vi "Lithographify.vi"(0 "interpolation distance":dbl, 1 "Path Settings.lvclass":refnum<class "Path Settings.lvclass">, 5 "Data In":cluster{string, cluster{"X":dbl, "Y":dbl}[]}, 7 "Direction":u16, 9 "Speed (um/s)":T1={"Schedule"=enum."Constant", "Settings"=variant(dbl 0.0)}, 11 "Voltage (V)":T1={"Schedule"=enum."Constant", "Settings"=variant(dbl 0.0)}, 13 "Enabled":bool) -> (4 "Lithography Data":T3)   [LabVIEW 2019]
doc: "This VI calculates the lithography data of one pattern and organizes it appropriately."
uses:
  typedefs/Schedule Types/Schedule--Formula.ctl
  Classes/Settings/ObjectSettings/ObjectSettings.lvclass
  Classes/Settings/Path Settings/Path Settings.lvclass
  typedefs/Schedule - enum.ctl
  typedefs/Voltage - cluster.ctl
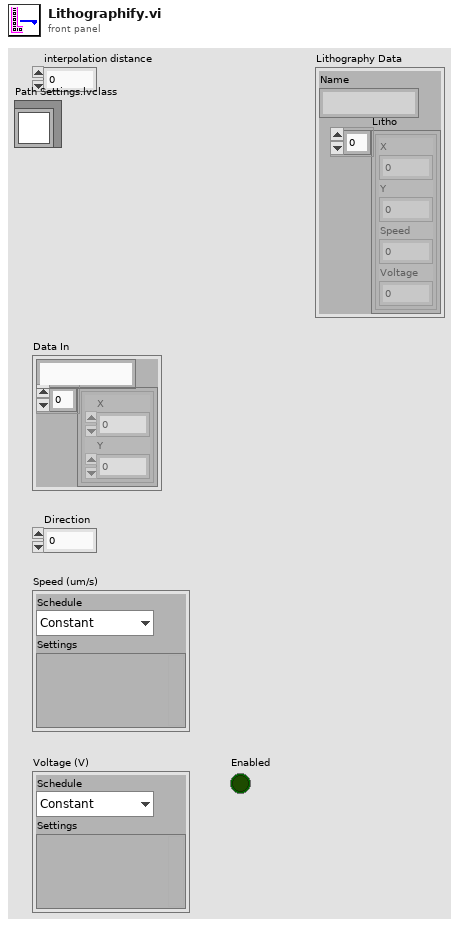
[diagram p1: front panel]
types:
  T1 = typedef "Voltage - cluster.ctl" = cluster{"Schedule":T2, "Settings":variant}
  T2 = typedef "Schedule - enum.ctl" = enum16{"Constant", "Ramp", "Fn. Generator", "Formula"}
  T3 = cluster{"Name":string, "Litho":cluster{"X":dbl, "Y":dbl, "Speed":dbl, "Voltage":dbl}[]}
  T4 = cluster{"X":dbl, "Y":dbl, "Speed":dbl, "Voltage":dbl}[]
  T5 = cluster{"X":dbl, "Y":dbl, "Speed":dbl, "Voltage":dbl}
  T6 = typedef "Schedule--Formula.ctl" = cluster{"formula":string, "formula length (nm)":dbl, "formula resolution (nm)":dbl}
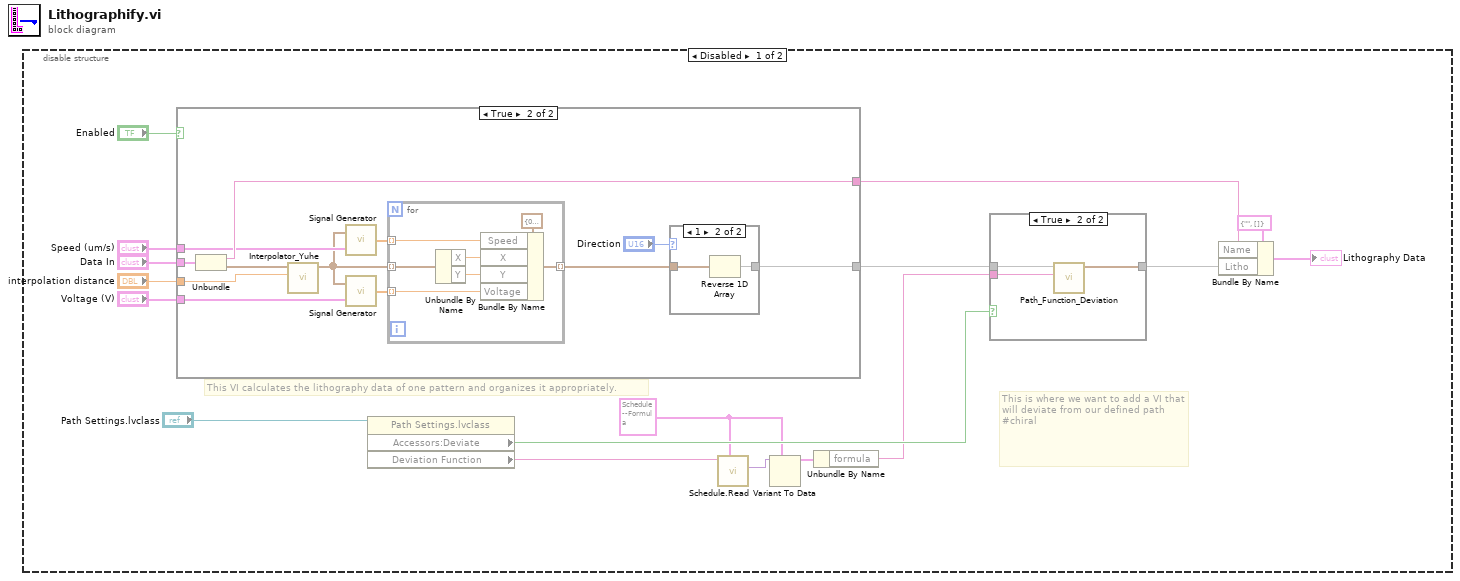
[diagram p0: block diagram]
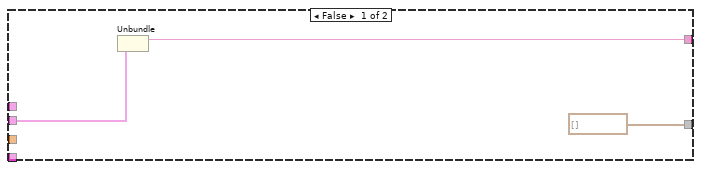
[diagram p3: hidden frame]
diagram:
  n1 = disable-structure shown="Disabled" {
    frame Disabled {
      w5 = T6 {"formula"="1*(step(170-t)*cos(0.62831853071*t)+step(t-170)*cos(0.62831853071*(t-170))*(-1))", "formula length (nm)"=340.0, "formula resolution (nm)"=0.001} ("Formula")
      # "This is where we want to add a VI that will deviate from our defined path\n#chiral"
      # "This VI calculates the lithography data of one pattern and organizes it appropriately."
      n2 = case shown="True" "Enabled" {
        tunnel: [w24 w36] -> w8
        tunnel: "Data In" -> [w22 w35]
        tunnel: "Voltage (V)" -> [_ w32]
        tunnel: "Speed (um/s)" -> [_ w31]
        tunnel: [T4 [] w29] -> w10
        tunnel: "interpolation distance" -> [_ w25]
        frame False {
          n3 = Unbundle(w22) -> (w24:string)  [unwired: 1 out]
        }
        frame True {
          n4 = Unbundle(w35) -> (w36:string, w27:cluster{"X":dbl, "Y":dbl}[])
          n5 = call "Interpolator_Yuhe.vi"("interpolation distance"=w25, "Array in"=w27) -> ("Array out"=w26:cluster{"X":dbl, "Y":dbl}[])  [unwired: 9 in]
          n6 = call "Signal Generator.vi"("Signal Properties"=w31, "Points"=w26) -> ("Signal"=w33:dbl[])
          n7 = call "Signal Generator.vi"("Signal Properties"=w32, "Points"=w26) -> ("Signal"=w34:dbl[])
          n8 = for {
            tunnel: w33 -> [w40] mode=indexing
            tunnel: w34 -> [w42] mode=indexing
            tunnel: w26 -> [w44] mode=indexing
            tunnel: [w41] -> w30 mode=indexing
            n9 = Unbundle By Name(w44) -> ("X"=w45:dbl, "Y"=w43:dbl)
            n10 = Bundle By Name(cluster=T5 {"X"=0.0, "Y"=0.0, "Speed"=0.0, "Voltage"=0.0} ("Litho Point"), "Speed"=w40, "X"=w45, "Y"=w43, "Voltage"=w42) -> (w41:T5)
          }
          n11 = case shown="1" "Direction" {
            tunnel: w30 -> [w37 w39]
            tunnel: [w37 w38] -> w29
            frame 0, Default {
            }
            frame 1 {
              n12 = Reverse 1D Array(array=w39) -> (reversed array=w38:T4)
            }
          }
        }
      }
      n13 = property class="Path Settings.lvclass"(reference="Path Settings.lvclass") -> ("Accessors:Deviate"=w6:bool, "Deviation Function"=w2:string)  [unwired: 1 in, 2 out]
      n14 = call "Schedule.Read.vi"("Data to Read"=w5, "Schedule <JSON> In"=w2) -> ("Data Out"=w4:variant)  [unwired: 7 in, 2 out]
      n15 = Variant To Data(type=w5, Variant=w4) -> (data=w3:T6)  [unwired: 1 in, 1 out]
      n16 = Unbundle By Name(w3) -> ("formula"=w1:string)
      n17 = case shown="True" w6 {
        tunnel: w10 -> [w18 w21]
        tunnel: [w18 w20] -> w9
        tunnel: w1 -> [_ w19]
        frame False {
        }
        frame True {
          n18 = call "Path_Function_Deviation.vi"("Function In"=w19, "Path Points In"=w21) -> ("Path Points Out"=w20:T4)  [unwired: 9 in]
        }
      }
      n19 = Bundle By Name(cluster=T3 {"Name"="", "Litho"=[]} ("Lithography Data"), "Name"=w8, "Litho"=w9) -> (→"Lithography Data":T3)
    }
    frame Enabled {
    }
  }
